vi "Enumerate Devices.vi"(8 "error in (no error)":errorcluster) -> (0 "error out":errorcluster, 3 "Devices":T1[](array[typedef]))   [LabVIEW 2020]
doc: "Enumerate the connected cameras."
uses:
  Device Enumeration.ctl
  bin/gindustrialcam_32-1.dll
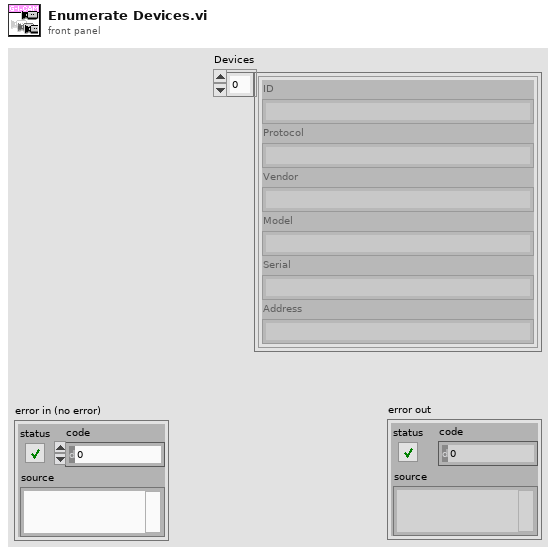
[diagram p1: front panel]
types:
  T1 = typedef "Device Enumeration.ctl" = cluster{"ID":string, "Protocol":string, "Vendor":string, "Model":string, "Serial":string, "Address":string}
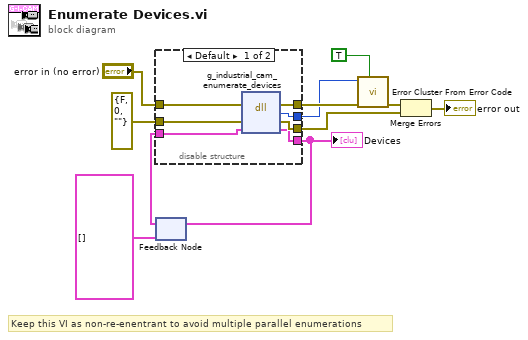
[diagram p0: block diagram]
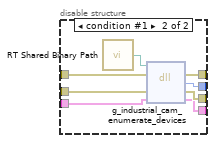
[diagram p2: hidden frame]
diagram:
  # "Keep this VI as non-re-enentrant to avoid multiple parallel enumerations"
  n1 = feedback #1(T1[] [] ("Array")) -> (w1:T1[])
  n2 = disable-structure shown="Default" {
    disable-tunnel: errorcluster {"status"=FALSE, "code"=0, "source"=""} ("error constant") -> [w18 w26]
    disable-tunnel: "error in (no error)" -> [w17 w25]
    disable-tunnel: [w16 w24] -> w9
    disable-tunnel: [w15 w23] -> w8
    disable-tunnel: [w14 w22] -> w5
    disable-tunnel: [w13 w21] -> w3
    disable-tunnel: w1 -> [w12 w20]
    frame condition #0 (active) {
      n3 = dll-call lib="C:/serenial/lib/g-industrial-camera/LabVIEW/g_industrial_cam/bin/gindustrialcam_*-1.*" fn="g_industrial_cam_enumerate_devices"(error in=w17, "Error"=w18, "Enumeration"=w12) -> (error out=w16:errorcluster, "MgError"=w15:i32, "Error"=w14:errorcluster, "Enumeration"=w13:T1[])  [unwired: 2 in, 1 out]
    }
    frame condition #1 {
      n4 = call "RT Shared Binary Path.vi"() -> ("Path"=w19:path)
      n5 = dll-call lib="?" fn="g_industrial_cam_enumerate_devices"(path in=w19, error in=w25, "Error"=w26, "Enumeration"=w20) -> (error out=w24:errorcluster, "MgError"=w23:i32, "Error"=w22:errorcluster, "Enumeration"=w21:T1[])  [unwired: 1 in, 1 out]
    }
  }
  "Devices" <- w3
  n6 = feedback-in #1(w3) -> ()
  n7 = call <vilib>:"Error Cluster From Error Code.vi"("show call chain? (False)"=TRUE, "error in (no error)"=w9, "error code (0)"=w8) -> ("error out"=w6:errorcluster)  [unwired: 6 in]
  n8 = Merge Errors(w6, w5) -> (→"error out":errorcluster)
